vi "CIVI Write.vi"(8 "error in":errorcluster, 10 "write buffer":string, 11 "VISA Session in":refnum<visa-resource-name>) -> (0 "error out":errorcluster, 3 "VISA Session out":refnum<visa-resource-name>)   [LabVIEW 2026]
doc: "Sends a SCPI command through an existing VISA session.\nAppends LF when needed using CIVI Ensure LF.vi.\nDoes not read a response or verify instrument acceptance.\nUse completion checking, readback and CIVI Error Query.vi\nas appropriate to verify the result.\nDoes not open or close the session."
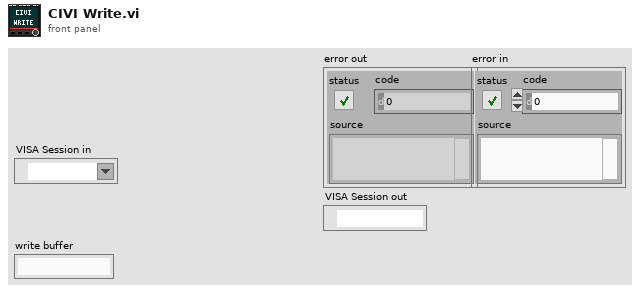
[diagram p1: front panel]
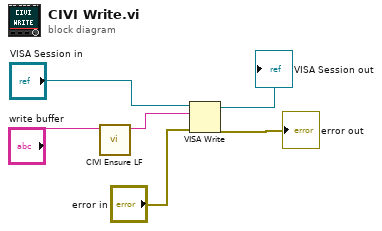
[diagram p0: block diagram]
diagram:
  n1 = call "CIVI Ensure LF.vi"("Command"="write buffer") -> ("Terminated Command"=w2:string)  [unwired: 10 in]
  n2 = VISA Write(VISA resource name="VISA Session in", write buffer=w2, error in (no error)="error in") -> (VISA resource name out=→"VISA Session out":refnum<visa-resource-name>, error out=→"error out":errorcluster)  [unwired: 1 out]
